vi "Read_Image.vi"(7 "PreProcessing_Options":T2={"DS_Name"="delete", "Input_Dims"={"C"=3, "H"=224, "W"=224}, "Cropping"={"Left"=0.0, "Top"=0.0, "Right"=1.0, "Bottom"=1.0}, "Interpolation Type"=1, "MultiStage_ReSample?"=FALSE, "Dataset_Stats"={"means"={"R"=0.5385, "G"=0.5348, "B"=0.551}, "stds"={"R"=0.3673, "G"=0.3673, "B"=0.3505}}} {"Dataset_Stats"."stds"."R" format="%#_3g"; "Dataset_Stats"."stds"."G" format="%#_3g"; "Dataset_Stats"."stds"."B" format="%#_3g"; "Dataset_Stats"."means"."R" format="%#_3g"; "Dataset_Stats"."means"."G" format="%#_3g"; "Dataset_Stats"."means"."B" format="%#_3g"; "Interpolation Type" items=["Zero Order", "Bi-Linear", "Quadratic", "Cubic Spline"]}, 8 "error in":errorcluster, 10 "IMAQ Name":string="train_orig", 11 "Img Path":path) -> (0 "error out":errorcluster, 1 "Image Out(Cropped)":T1, 2 "Image Out (Preproc)":T1, 3 "Image Out (Preproc)":sgl[][][](array[numeric]), 4 "Image Out(Orig)":T1, 5 "dT_Img_Read":dbl=0.005897299968637526 format="%#_6p")   [LabVIEW 2020]
uses:
  <vilib>/Ngene/DeepLTK Anomaly Detection Addon/Toolkit/API/Controls/NNPC_PreProcessing_Options.ctl
  <vilib>/Ngene/Deep Learning Toolkit/Toolkit/NN_Data/API/NN_Dims(C,H,W).ctl
  <vilib>/Ngene/DeepLTK Anomaly Detection Addon/Toolkit/API/Controls/Crop_CFG.ctl
  <vilib>/Ngene/DeepLTK Anomaly Detection Addon/Toolkit/API/Controls/NNPC_DS_Stats.ctl
  <vilib>/Ngene/DeepLTK Anomaly Detection Addon/Toolkit/API/Controls/Image_Stats_RGB.ctl
  <vilib>/vision/Image Controls.llb/IMAQ Image.ctl
  e27f082d-ee3a-42c8-8c3d-01a79e3cbb58.vi
  addfa468-52d3-4960-9c35-afb1bd2196bd.vi
  <vilib>/Utility/High Resolution Relative Seconds.vi
  <vilib>/Ngene/DeepLTK Anomaly Detection Addon/Toolkit/DeepLTK_Anomaly_Detection_Addon.lvlib
  <vilib>/Ngene/Deep Learning Toolkit/Toolkit/Deep_Learning_Toolkit_by_Ngene.lvlib
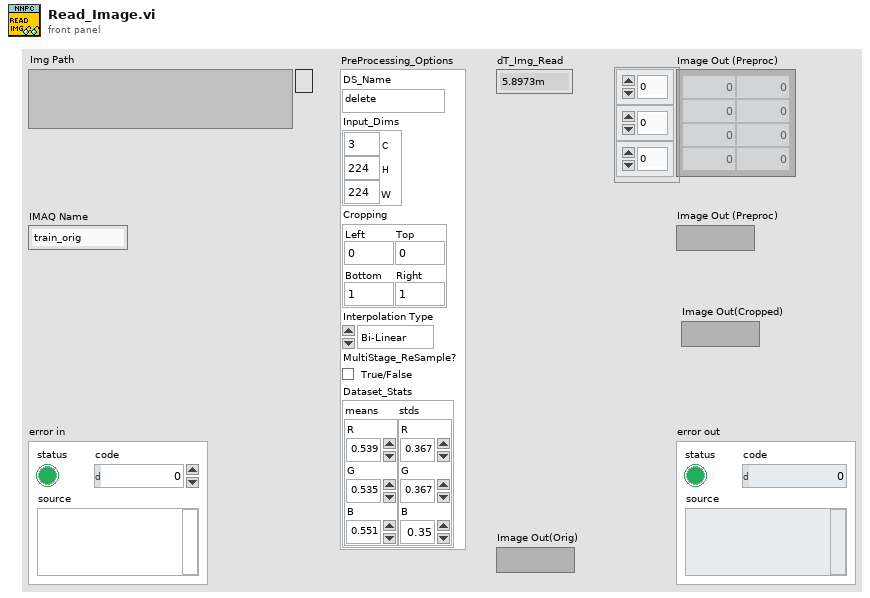
[diagram p1: front panel]
types:
  T1 = typedef "IMAQ Image.ctl" = refnum<image>
  T2 = typedef "DeepLTK_Anomaly_Detection_Addon.lvlib/NNPC_PreProcessing_Options.ctl" = cluster{"DS_Name":string, "Input_Dims":T3, "Cropping":T4, "Interpolation Type":u32, "MultiStage_ReSample?":bool, "Dataset_Stats":T5}
  T3 = typedef "Deep_Learning_Toolkit_by_Ngene.lvlib/NN_Dims(C,H,W).ctl" = cluster{"C":i32, "H":i32, "W":i32}
  T4 = typedef "DeepLTK_Anomaly_Detection_Addon.lvlib/Crop_CFG.ctl" = cluster{"Left":sgl, "Top":sgl, "Right":sgl, "Bottom":sgl}
  T5 = typedef "DeepLTK_Anomaly_Detection_Addon.lvlib/NNPC_DS_Stats.ctl" = cluster{"means":T6, "stds":T6}
  T6 = typedef "DeepLTK_Anomaly_Detection_Addon.lvlib/Image_Stats_RGB.ctl" = cluster{"R":sgl, "G":sgl, "B":sgl}
  T7 = typedef "Image Type" = u32
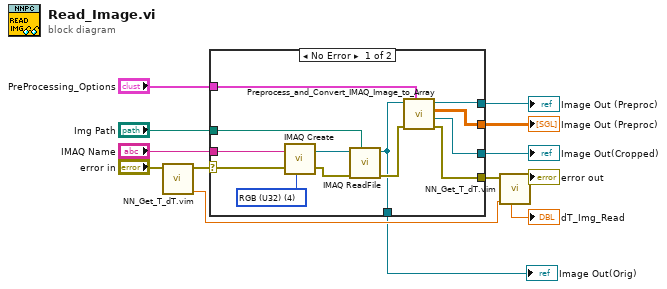
[diagram p0: block diagram]
diagram:
  n1 = call "NN_Get_T_dT.vim"("error in"="error in") -> ("T_out"=w6:dbl, "error out"=w9:errorcluster)  [unwired: 6 in, 1 out]
  n2 = case shown="No Error" w9 {
    selector: w9 -> [w23 w27]
    tunnel: "Img Path" -> [w25 _]
    tunnel: [w18 _] -> w11
    tunnel: [w24 w27] -> w10
    tunnel: "IMAQ Name" -> [w20 _]
    tunnel: [w17 _] -> w3
    tunnel: "PreProcessing_Options" -> [w16 _]
    tunnel: [w15 _] -> w2
    tunnel: [w14 _] -> w1
    frame No Error {
      w21 = T7 4 items=["Grayscale (U8)", "Grayscale (I16)", "Grayscale (SGL)", "Complex (CSG)", "RGB (U32)", "HSL (U32)", "RGB (U64)", "Grayscale (U16)"] ("Image Type")
      n3 = call "IMAQ Create"("Image Name"=w20, "Image Type"=w21, "error in (no error)"=w23) -> ("New Image"=w26:T1, "error out"=w19:errorcluster)  [unwired: 2 in]
      n4 = call "IMAQ ReadFile"("File Path"=w25, "error in (no error)"=w19, "Image"=w26) -> ("error out"=w22:errorcluster, "Image Out"=w14:T1)  [unwired: 4 in, 3 out]
      n5 = call "Preprocess_and_Convert_IMAQ_Image_to_Array.vi"("PreProcessing_Options"=w16, "error in (no error)"=w22, "Image In"=w14) -> ("error out"=w24:errorcluster, "Image_Out(Cropped)"=w15:T1, "Norm_Img_Out"=w18:sgl[][][], "Image_Out(PreProcessed)"=w17:T1)  [unwired: 4 in, 1 out]
    }
    frame Error {
    }
  }
  "Image Out (Preproc)" <- w11
  "Image Out (Preproc)" <- w3
  "Image Out(Cropped)" <- w2
  "Image Out(Orig)" <- w1
  n6 = call "NN_Get_T_dT.vim"("T_in"=w6, "error in"=w10) -> ("error out"=→"error out":errorcluster, "dT"=→"dT_Img_Read":dbl)  [unwired: 5 in, 1 out]
